vi "VIH HelpGen - Build Control Description Table.vi"(4 "InstanceRef":string, 5 "HTML Folder":path, 6 "Ctrl Dscr Params":T5, 7 "Image Folder":path, 8 "error in":errorcluster, 9 "Table Templates":T7, 10 "Ctrl Attributes":T6[](array[typedef]), 11 "Ctrl refnums":refnum<vi>[](array[refnum])) -> (0 "error out":errorcluster, 2 "HTML out":string, 3 "dup Ctrl refnums":refnum<vi>[](array[refnum]))   [LabVIEW 2014]
doc: "::: VI Helpeks :::\nCopyright (c) 2000-2026 Konstantin Shifershteyn. All rights reserved."
uses:
  VIH HelpGen Typedef - Table Templates Cluster - VI Help.ctl
  VIH HelpGen Typedef - Control Terminal Attributes Cluster.ctl
  VIH HelpGen Typedef - Cluster - Control Rule.ctl
  VIH HelpGen Typedef - Enum - Description Mode.ctl
  VIH HelpGen Typedef - Enum - Default,Enable,Disable.ctl
  VIH HelpGen Typedef - Cluster - Enum Value Info.ctl
panel:
  # "VI Helpeks\nCopyright (c) 2012-2026 Konstantin Shifershteyn"
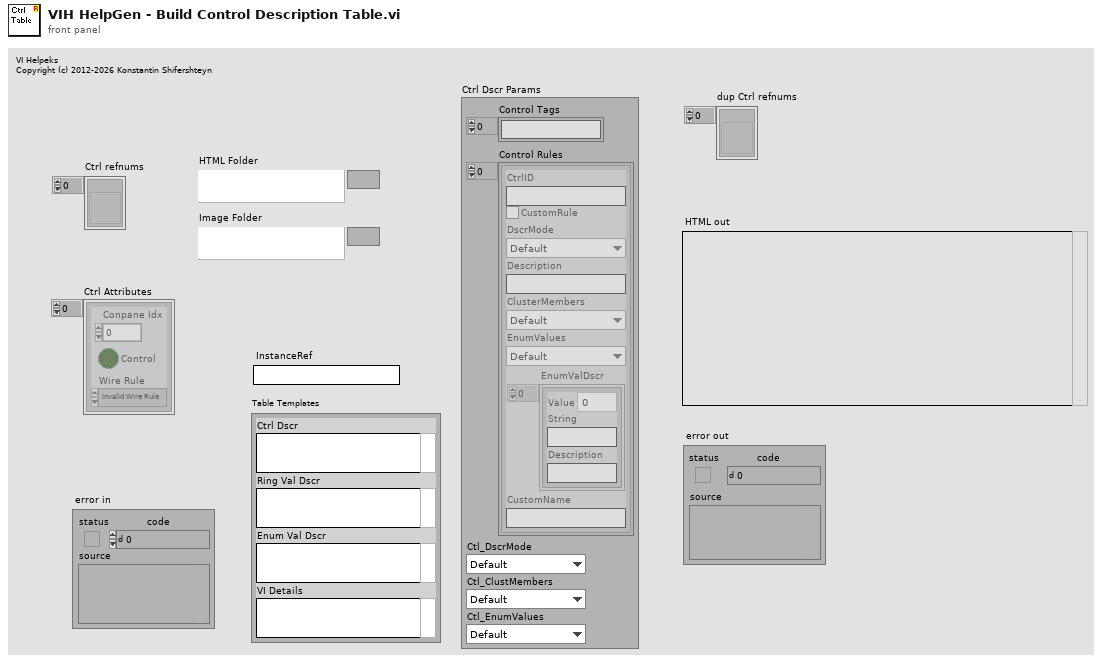
[diagram p1: front panel]
types:
  T1 = typedef "VIH HelpGen Typedef - Cluster - Control Rule.ctl" = cluster{"CtrlID":string, "CustomRule":bool, "DscrMode":T2, "Description":string, "ClusterMembers":T3, "EnumValues":T3, "EnumValDscr":T4[], "CustomName":string}
  T2 = typedef "VIH HelpGen Typedef - Enum - Description Mode.ctl" = enum16{"Default", "Description", "Description1", "Description2", "Custom", "None"}
  T3 = typedef "VIH HelpGen Typedef - Enum - Default,Enable,Disable.ctl" = enum16{"Default", "Enable", "Disable"}
  T4 = typedef "VIH HelpGen Typedef - Cluster - Enum Value Info.ctl" = cluster{"Value":ext, "String":string, "Description":string}
  T5 = cluster{"Control Tags":string[], "Control Rules":T1[], "Ctl_DscrMode":T2, "Ctl_ClustMembers":T3, "Ctl_EnumValues":T3}
  T6 = typedef "VIH HelpGen Typedef - Control Terminal Attributes Cluster.ctl" = cluster{"Conpane Idx":i32, "Control":bool, "Wire Rule":enum16{"Invalid Wire Rule", "Required", "Recommended", "Optional", "Dynamic Dispatch"}}
  T7 = typedef "VIH HelpGen Typedef - Table Templates Cluster - VI Help.ctl" = cluster{"Ctrl Dscr":string, "Ring Val Dscr":string, "Enum Val Dscr":string, "VI Details":string}
  T8 = typedef "imagedata.ctl" = cluster{"image type":i32, "image depth":i32, "image":u8[], "mask":u8[], "colors":u32[], "Rectangle":cluster{"left":i16, "top":i16, "right":i16, "bottom":i16}}
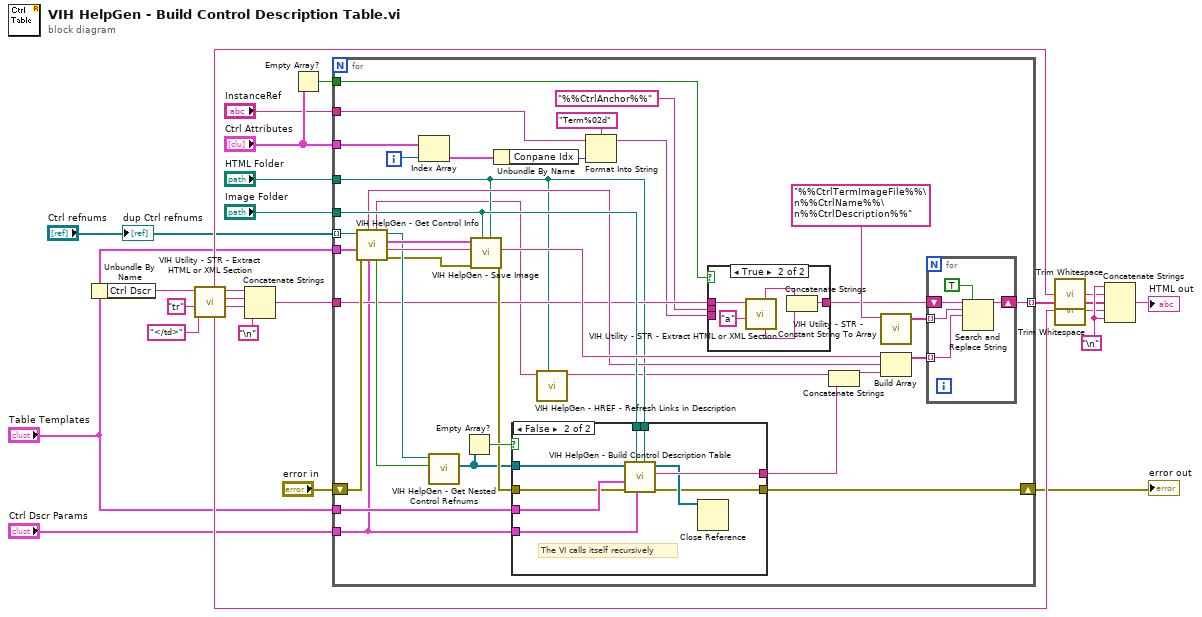
[diagram p0: block diagram]
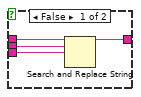
[diagram p2: hidden frame]
diagram:
  w12 = "\n"
  n1 = Unbundle By Name("Table Templates") -> ("Ctrl Dscr"=w10:string)
  n2 = call "VIH Utility - STR - Extract HTML or XML Section.vi"("Contain (opt)"="</td>", "Section name"="tr", "HTML in"=w10) -> ("end"=w22:string, "body"=w23:string, "start"=w24:string, "after"=w20:string, "before"=w19:string)  [unwired: 4 in]
  n3 = Concatenate Strings(w24, w23, w22, "\n") -> (w21:string)
  n4 = Empty Array?(array="Ctrl Attributes") -> (empty?=w4:bool)
  n5 = for {
    tunnel: w21 -> [w34]
    tunnel: "Ctrl refnums" -> [w62] mode=indexing
    tunnel: "Image Folder" -> [w57]
    tunnel: "HTML Folder" -> [w29]
    shift-right: [w53] -> w14
    shift-left: "error in" -> [w45]
    tunnel: "Table Templates" -> [w55]
    tunnel: "Table Templates" -> [w43]
    tunnel: [w36] -> w8 mode=indexing
    tunnel: "Ctrl Attributes" -> [w41]
    tunnel: w4 -> [w32]
    tunnel: "Ctrl Dscr Params" -> [w30]
    tunnel: "InstanceRef" -> [w26]
    i -> [w40]
    n6 = call "VIH HelpGen - Get Control Info.vi"("Ctrl Dscr Params"=w30, "error in"=w45, "Table Templates"=w43, "Ctl Refnum"=w62) -> ("error out"=w44:errorcluster, "Image Filename"=w58:string, "Ctrl Term Image"=w59:T8, "dup Ctl Refnum"=w50:refnum<vi>, "Show members"=w46:bool, "Ctrl Description"=w28:string, "Ctrl Name"=w42:string)  [unwired: 1 in]
    n7 = Index Array(array=w41, index=w40) -> (element=w37:T6)
    n8 = call "VIH HelpGen - Get Nested Control Refnums.vi"("Get members (T)"=w46, "Ctl Refnum"=w50) -> ("Ctl Refnums"=w49:refnum<vi>[])  [unwired: 7 in, 2 out]
    n9 = Empty Array?(array=w49) -> (empty?=w56:bool)
    n10 = call "VIH HelpGen - Save Image.vi"("HTML Folder"=w29, "Image Folder"=w57, "error in"=w44, "Image Filename"=w58, "image data"=w59) -> ("error out"=w54:errorcluster, "path for HTML"=w60:string)  [unwired: 4 in, 1 out]
    n11 = Unbundle By Name(w37) -> ("Conpane Idx"=w39:i32)
    n12 = case shown="False" w56 {
      tunnel: [_ w76] -> w51
      tunnel: w55 -> [_ w81]
      tunnel: w57 -> [_ w78]
      tunnel: w29 -> [_ w77]
      tunnel: w49 -> [_ w79]
      tunnel: w54 -> [w72 w80]
      tunnel: [w72 w74] -> w53
      tunnel: w30 -> [_ w73]
      frame True {
      }
      frame False {
        # "The VI calls itself recursively"
        n13 = call "VIH HelpGen - Build Control Description Table.vi"("HTML Folder"=w77, "Ctrl Dscr Params"=w73, "Image Folder"=w78, "error in"=w80, "Table Templates"=w81, "Ctrl refnums"=w79) -> ("error out"=w74:errorcluster, "HTML out"=w76:string, "dup Ctrl refnums"=w75:refnum<vi>[])  [unwired: 3 in]
        n14 = Close Reference(reference=w75) -> ()  [unwired: 1 in, 1 out]
      }
    }
    n15 = call "VIH HelpGen - HREF - Refresh Links in Description.vi"("HTML Folder"=w29, "Description in"=w28) -> ("Description out"=w27:string)  [unwired: 9 in]
    n16 = Format Into String(format string="Term%02d", initial string=w26, w39) -> (resulting string=w33:string)  [unwired: 1 in, 1 out]
    n17 = case shown="True" w32 {
      tunnel: w34 -> [w66 w71]
      tunnel: [w65 w67] -> w35
      tunnel: "%%CtrlAnchor%%" -> [w64 _]
      tunnel: w33 -> [w63 _]
      frame False {
        n18 = Search and Replace String(input string=w66, search string=w64, replace string=w63) -> (result string=w65:string)  [unwired: 5 in, 3 out]
      }
      frame True {
        n19 = call "VIH Utility - STR - Extract HTML or XML Section.vi"("Section name"="a", "HTML in"=w71) -> ("after"=w68:string, "before"=w69:string)  [unwired: 5 in, 3 out]
        n20 = Concatenate Strings(w69, w68) -> (w67:string)
      }
    }
    n21 = Concatenate Strings(w27, w51) -> (w52:string)
    n22 = call "VIH Utility - STR - Constant String To Array.vi"("String in"="%%CtrlTermImageFile%%\n%%CtrlName%%\n%%CtrlDescription%%") -> ("Array out"=w48:string[])  [unwired: 10 in]
    n23 = Build Array(w60, w42, w52) -> (w61:string[])
    n24 = for {
      shift-right: [w85] -> w36
      shift-left: w35 -> [w86]
      tunnel: w48 -> [w83] mode=indexing
      tunnel: w61 -> [w82] mode=indexing
      n25 = Search and Replace String(replace all?=TRUE, input string=w86, search string=w83, replace string=w82) -> (result string=w85:string)  [unwired: 4 in, 3 out]
    }
  }
  "error out" <- w14
  n26 = call <vilib>:"Trim Whitespace.vi"("string"=w19) -> ("trimmed string"=w7:string)  [unwired: 1 in]
  n27 = call <vilib>:"Trim Whitespace.vi"("string"=w20) -> ("trimmed string"=w6:string)  [unwired: 1 in]
  n28 = Concatenate Strings(w12, w7, w8, w6, w12) -> (→"HTML out":string)
  "dup Ctrl refnums" <- "Ctrl refnums"
